vi "Alerte min-max temperature.vi"() -> ()   [LabVIEW 2022 SP3]
uses:
  Enum/Enum 2.ctl
  Variables globales/Variables glob EUROTHERM.vi
  Variables globales/Variable glob Th.vi
  Variables globales/Variable glob Pt.vi
  Variables globales/Variable glob alertes min-max temperatures.vi
panel:
  out "Nb pages":u8
  in  "ajouter":bool
  in  "Groupes":T1(array[cluster])=[{"Temperature min (°C)"=-10.0, "Temperature max (°C)"=80.0, "Alerte"=FALSE, "Capteurs a controler"=[5], "N°"=0}] caption="Groupes alertes min-max températures" {"Temperature max (°C)" format="%.2f"; "Temperature min (°C)" format="%.2f"}
  in  "OK":bool
  in  "Annuler":bool
  # "PARAMeTRES POUR ALERTE Min max TEMPeRATURE PAR ENVOI D'UN MAIL"
  # "Ce logiciel et les informations qu'il contient, sont la propriété de l’IAS et ne peuvent être diffusés sans l’autorisation de la Station d’étalonnage"
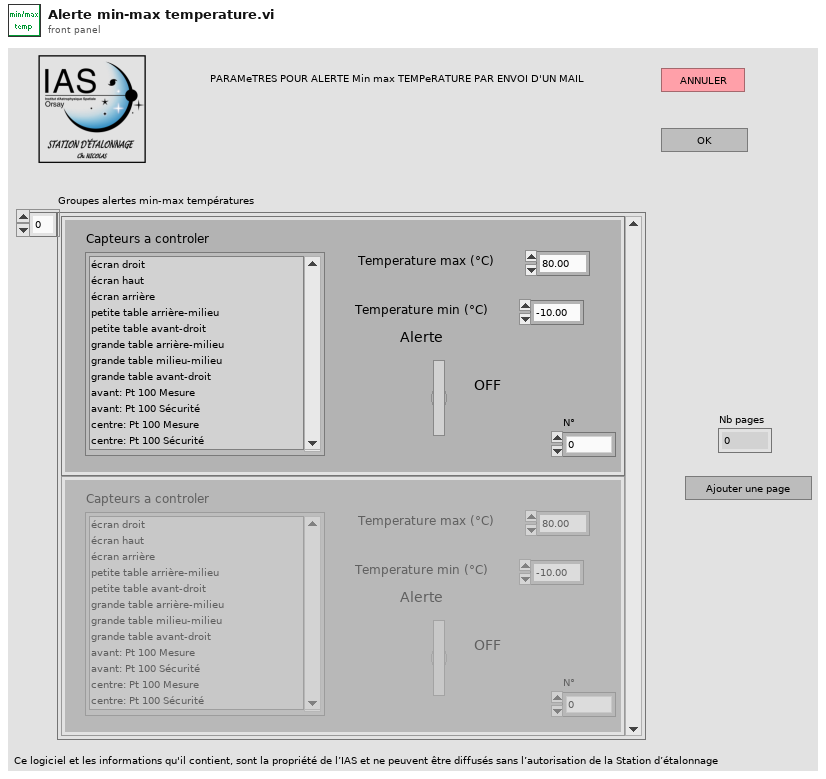
[diagram p1: front panel]
types:
  T1 = cluster{"Temperature min (°C)":dbl, "Temperature max (°C)":dbl, "Alerte":bool, "Capteurs a controler":i32[], "N°":u16}[]
  T2 = typedef "Enum 2.ctl" = enum16{"init noms", "initialisation", "choix", "GO"}
  T3 = cluster{"Noms voies select acqui 1COM":string[]}[]
  T4 = cluster{"Nom tache Pt":refnum<k21>, "Noms des Pt":string[], "Nb Pt":i16, "Selection Pt":bool[], "Nom Pt selectionnees":string[]}[]
  T5 = cluster{"Nom tache Th":refnum<k21>, "Noms des Th":string[], "Nb Th":i16, "Selection Th":bool[], "Nom Th selectionnes":string[]}[]
  T6 = cluster{"Alerte temp min/max":bool, "température max":dbl, "température min":dbl, "Défaut min/max temp":bool, "Indices à controler":i16[], "N°":u16}[]
  T7 = cluster{"Temperature min (°C)":dbl, "Temperature max (°C)":dbl, "Alerte":bool, "Capteurs a controler":i32[], "N°":u16}
  T8 = cluster{"Alerte temp min/max":bool, "température max":dbl, "température min":dbl, "Défaut min/max temp":bool, "Indices à controler":i16[], "N°":u16}
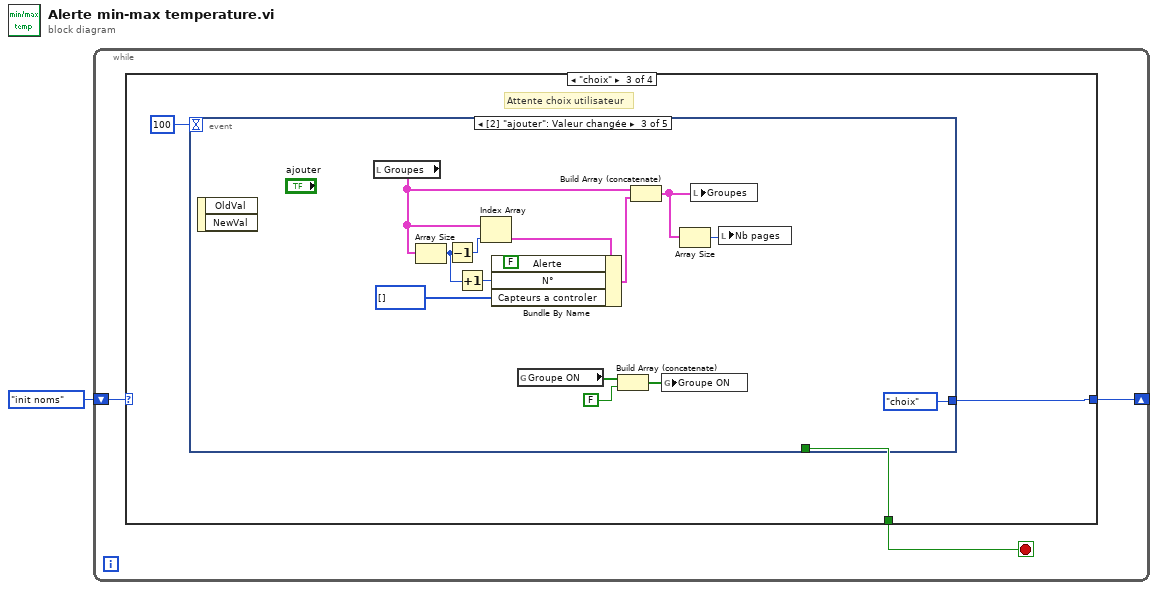
[diagram p0: block diagram]
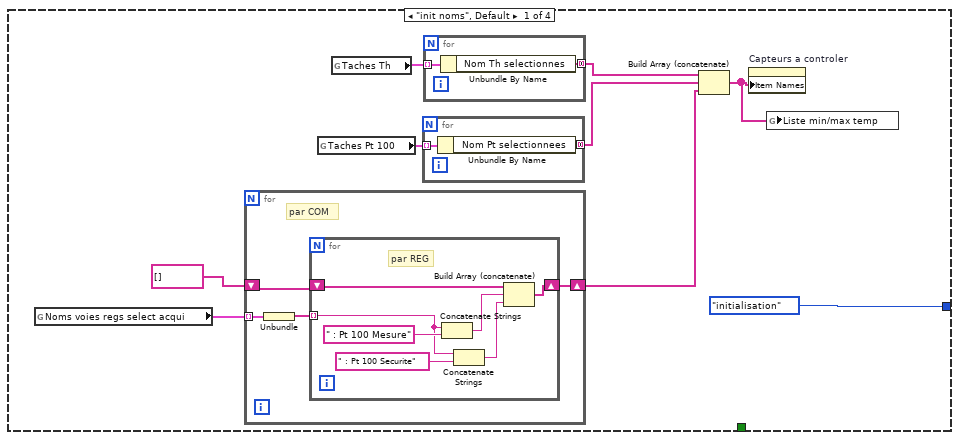
[diagram p2: hidden frame]
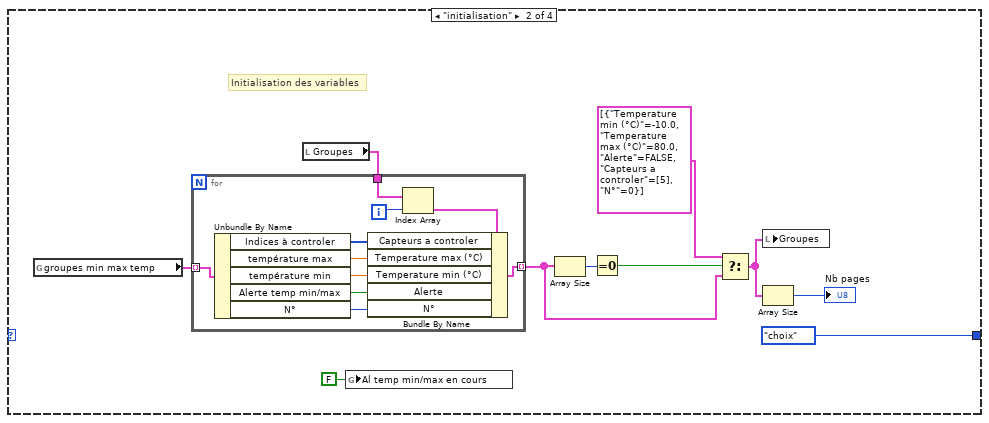
[diagram p3: hidden frame]
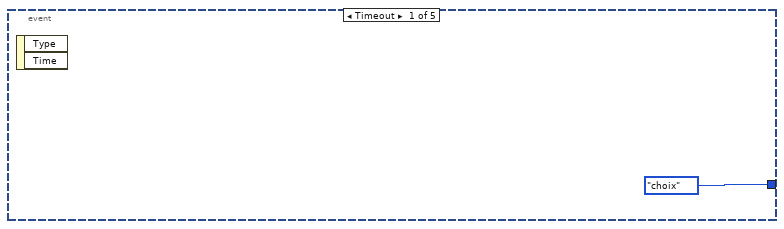
[diagram p4: hidden frame]
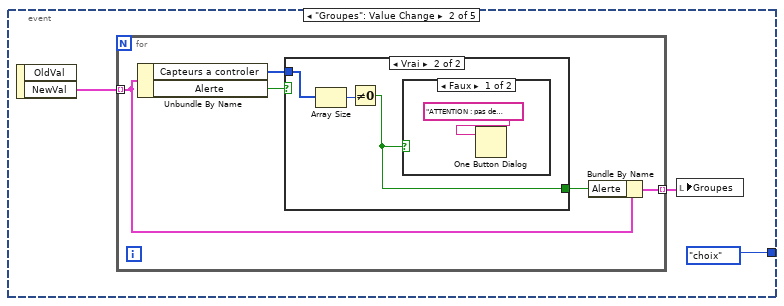
[diagram p5: hidden frame]
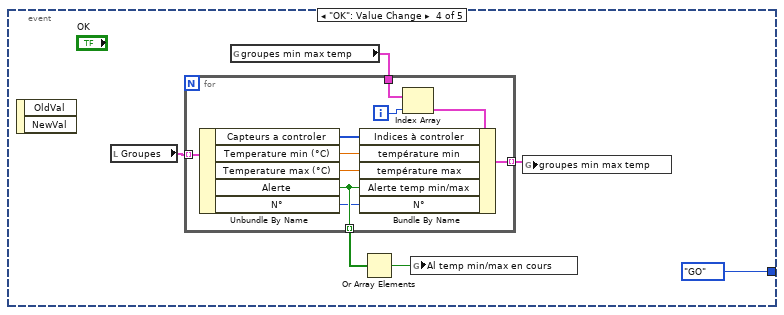
[diagram p8: hidden frame]
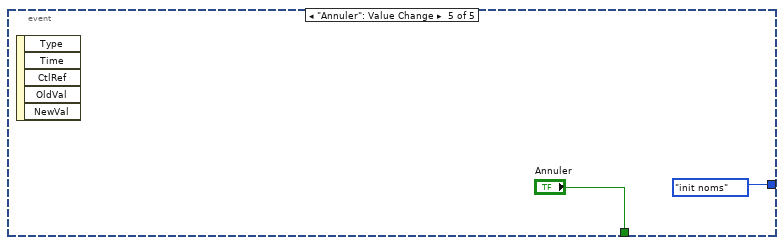
[diagram p9: hidden frame]
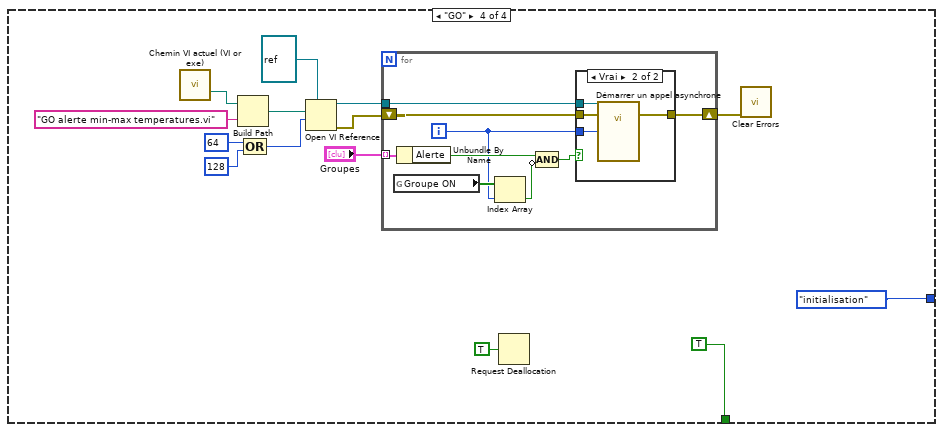
[diagram p10: hidden frame]
diagram:
  n1 = while {
    shift-right: [w3] -> _
    shift-left: Enum_2."init noms" ("Énum") -> [w4]
    stop <- w2 stop-if-true
    n2 = case shown="\"choix\"" w4 {
      tunnel: [Enum_2."initialisation" ("Énum") Enum_2."choix" ("Énum") w50 Enum_2."initialisation" ("Énum")] -> w3
      tunnel: [_ _ w49 TRUE] -> w2
      frame "init noms", Default {
        n3 = global read "Variables glob EUROTHERM.vi" "Noms voies regs select acqui"() -> (w12:T3)
        n4 = for {
          tunnel: w12 -> [w20] mode=indexing
          shift-right: [w21] -> w6
          shift-left: string[] [] -> [w18]
          # "par COM"
          n5 = Unbundle(w20) -> ("Noms voies select acqui 1COM"=w19:string[])
          n6 = for {
            tunnel: w19 -> [w23] mode=indexing
            shift-right: [w24] -> w21
            shift-left: w18 -> [w28]
            # "par REG"
            n7 = Concatenate Strings(w23, " : Pt 100 Mesure") -> (w25:string)
            n8 = Concatenate Strings(w23, " : Pt 100 Securite") -> (w22:string)
            n9 = Build Array (concatenate)(w28, w25, w22) -> (w24:string[])
          }
        }
        n10 = global read "Variable glob Pt.vi" "Taches Pt 100"() -> (w7:T4)
        n11 = global read "Variable glob Th.vi" "Taches Th"() -> (w10:T5)
        n12 = for {
          tunnel: w7 -> [w17] mode=indexing
          tunnel: [w16] -> w8 mode=concatenating
          n13 = Unbundle By Name(w17) -> ("Nom Pt selectionnees"=w16:string[])
        }
        n14 = for {
          tunnel: w10 -> [w15] mode=indexing
          tunnel: [w14] -> w9 mode=concatenating
          n15 = Unbundle By Name(w15) -> ("Nom Th selectionnes"=w14:string[])
        }
        n16 = Build Array (concatenate)(w9, w8, w6) -> (w5:string[])
        n17 = property on="Capteurs a controler" class="LstDér (strict)"("Item Names"=w5) -> ()  [unwired: 2 in, 2 out]
        n18 = global write "Variable glob alertes min-max temperatures.vi" "Liste min/max temp"(w5) -> ()
      }
      frame "initialisation" {
        # "Initialisation des variables"
        n19 = global read "Variable glob alertes min-max temperatures.vi" "groupes min max temp"() -> (w37:T6)
        n20 = local read "Groupes"() -> (w36:T1)
        n21 = for {
          tunnel: w37 -> [w48] mode=indexing
          tunnel: w36 -> [w47]
          tunnel: [w40] -> w33 mode=indexing
          i -> [w46]
          n22 = Unbundle By Name(w48) -> ("Indices à controler"=w44:i16[], "température max"=w43:dbl, "température min"=w42:dbl, "Alerte temp min/max"=w41:bool, "N°"=w39:u16)
          n23 = Index Array(array=w47, index=w46) -> (element=w45:T7)
          n24 = Bundle By Name(cluster=w45, "Capteurs a controler"=w44, "Temperature max (°C)"=w43, "Temperature min (°C)"=w42, "Alerte"=w41, "N°"=w39) -> (w40:T7)
        }
        n25 = global write "Variable glob alertes min-max temperatures.vi" "Al temp min/max en cours"(FALSE ("Al temp min/max en cours")) -> ()
        n26 = Array Size(array=w33) -> (size(s)=w34:i32)
        n27 = Equal To 0?(x=w34) -> (x = 0?=w35:bool)
        n28 = Select(t=T1 [{"Temperature min (°C)"=-10.0, "Temperature max (°C)"=80.0, "Alerte"=FALSE, "Capteurs a controler"=[5], "N°"=0}] ("cas vrai"), s=w35, f=w33) -> (s? t:f=w31:T1)
        n29 = local write "Groupes"(w31) -> ()
        n30 = Array Size(array=w31) -> (size(s)=→"Nb pages":i32)
      }
      frame "choix" {
        # "Attente choix utilisateur"
        n31 = event shown="[2] \"ajouter\": Valeur changée" {
          selector: _ -> [_ _ _ _ _]
          dyn-events: _ -> [_ _ _ _ _]
          timeout: 100 -> [_ _ _ _ _]
          tunnel: [Enum_2."choix" ("Énum") Enum_2."choix" ("Énum") Enum_2."choix" ("Énum") Enum_2."GO" ("Énum") Enum_2."init noms" ("Énum")] -> w50
          tunnel: [_ _ _ _ "Annuler"] -> w49
          event Timeout {
            n32 = event-data() -> ()  [unwired: 1 in, 2 out]
          }
          event "Groupes": Value Change {
            n33 = event-data() -> ("NewVal"=w54:T1)  [unwired: 1 in, 1 out]
            n34 = for {
              tunnel: w54 -> [w59] mode=indexing
              tunnel: [w56] -> w53 mode=indexing
              n35 = Unbundle By Name(w59) -> ("Capteurs a controler"=w58:i32[], "Alerte"=w60:bool)
              n36 = case shown="Vrai" w60 {
                selector: w60 -> [w61 _]
                tunnel: w58 -> [_ w64]
                tunnel: [w61 w62] -> w57
                frame False {
                }
                frame True {
                  n37 = Array Size(array=w64) -> (size(s)=w63:i32)
                  n38 = Not Equal To 0?(x=w63) -> (x != 0?=w62:bool)
                  n39 = case shown="Faux" w62 {
                    frame False {
                      n40 = One Button Dialog(message="ATTENTION : pas de capteur choisi dans la liste") -> ()  [unwired: 1 in, 1 out]
                    }
                    frame True {
                    }
                  }
                }
              }
              n41 = Bundle By Name(cluster=w59, "Alerte"=w57) -> (w56:T7)
            }
            n42 = local write "Groupes"(w53) -> ()
          }
          event "ajouter": Value Change {
            n43 = event-data() -> ()  [unwired: 1 in, 2 out]
            n44 = local read "Groupes"() -> (w76:T1)
            n45 = Array Size(array=w76) -> (size(s)=w68:i32)
            n46 = Decrement(x=w68) -> (x-1=w75:i32)
            n47 = Increment(x=w68) -> (x+1=w67:i32)
            n48 = Index Array(array=w76, index=w75) -> (element=w77:T7)
            n49 = Bundle By Name(cluster=w77, "Alerte"=FALSE, "N°"=w67, "Capteurs a controler"=i32[] []) -> (w79:T7)
            n50 = global read "Variable glob alertes min-max temperatures.vi" "Groupe ON"() -> (w71:bool[])
            n51 = Build Array (concatenate)(w71, FALSE ("Alerte")) -> (w69:bool[])
            n52 = Build Array (concatenate)(w76, w79) -> (w73:T1)
            n53 = global write "Variable glob alertes min-max temperatures.vi" "Groupe ON"(w69) -> ()
            n54 = Array Size(array=w73) -> (size(s)=w72:i32)
            n55 = local write "Groupes"(w73) -> ()
            n56 = local write "Nb pages"(w72) -> ()
          }
          event "OK": Value Change {
            n57 = event-data() -> ()  [unwired: 1 in, 2 out]
            n58 = local read "Groupes"() -> (w83:T1)
            n59 = global read "Variable glob alertes min-max temperatures.vi" "groupes min max temp"() -> (w82:T6)
            n60 = for {
              tunnel: w83 -> [w95] mode=indexing
              tunnel: w82 -> [w94]
              tunnel: [w89] -> w81 mode=indexing
              tunnel: [w87] -> w84 mode=indexing
              i -> [w93]
              n61 = Unbundle By Name(w95) -> ("Capteurs a controler"=w91:i32[], "Temperature min (°C)"=w90:dbl, "Temperature max (°C)"=w88:dbl, "Alerte"=w87:bool, "N°"=w86:u16)
              n62 = Index Array(array=w94, index=w93) -> (element=w92:T8)
              n63 = Bundle By Name(cluster=w92, "Indices à controler"=w91, "température min"=w90, "température max"=w88, "Alerte temp min/max"=w87, "N°"=w86) -> (w89:T8)
            }
            n64 = Or Array Elements(Boolean array=w84) -> (logical OR=w80:bool)
            n65 = global write "Variable glob alertes min-max temperatures.vi" "Al temp min/max en cours"(w80) -> ()
            n66 = global write "Variable glob alertes min-max temperatures.vi" "groupes min max temp"(w81) -> ()
          }
          event "Annuler": Value Change {
            n67 = event-data() -> ()  [unwired: 1 in, 5 out]
          }
        }
      }
      frame "GO" {
        n68 = call "Chemin VI actuel (VI or exe).vi"() -> ("VI or executable installation directory"=w104:path)  [unwired: 14 in, 1 out]
        n69 = Build Path(base path=w104, name or relative path="GO alerte min-max temperatures.vi" ("nom ou chemin relatif")) -> (appended path=w99:path)
        n70 = Compound Arithmetic op=OR(64 ("options"), 128 ("options")) -> (w103:i32)
        n71 = Open VI Reference(type specifier VI Refnum (for type only)=refnum<vi> refnum ("spécificateur de type du refnum de VI (pour type seulement)"), vi path=w99, options=w103) -> (vi reference=w105:refnum<vi>, error out=w106:errorcluster)  [unwired: 3 in]
        n72 = for {
          shift-right: [w119] -> w108
          shift-left: w106 -> [w120]
          tunnel: w105 -> [w118]
          tunnel: "Groupes" -> [w117] mode=indexing
          i -> [w113]
          n73 = global read "Variable glob alertes min-max temperatures.vi" "Groupe ON"() -> (w114:bool[])
          n74 = Unbundle By Name(w117) -> ("Alerte"=w116:bool)
          n75 = Index Array(array=w114, index=w113) -> (element=w112:bool)
          n76 = Compound Arithmetic op=AND ("Opérateur arithmétique")(w116, invert w112) -> (w115:bool)
          n77 = case shown="Vrai" w115 {
            tunnel: w120 -> [w121 w125]
            tunnel: [w121 w124] -> w119
            tunnel: w118 -> [_ w123]
            tunnel: w113 -> [_ w122]
            frame False {
            }
            frame True {
              n78 = call-by-ref "Démarrer un appel asynchrone"(reference=w123, error in=w125, "Numéro"=w122) -> (error out=w124:errorcluster)  [unwired: 2 in, 2 out]
            }
          }
        }
        n79 = Request Deallocation(TRUE ("flag")) -> ()
        n80 = call <vilib>:"Clear Errors.vi"("error in (no error)"=w108) -> ()  [unwired: 5 in, 2 out]
      }
    }
  }
